vi "Get Context.vi"(8 "error in":errorcluster) -> (0 "error out":errorcluster, 3 "context":refnum<class "zmq_context.lvclass">)   [LabVIEW 2019, in "RemoteControl.ZMQ.lvlib" / "ZMQ.ContextManager.lvlib"]
uses:
  ZMQ.ContextManager.lvlib
  <vilib>/addons/zeromq/zmq_context.lvclass
  Typedefs/Action--enum.ctl
  private/Context Owner.vi
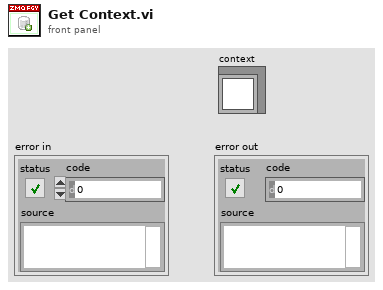
[diagram p1: front panel]
types:
  T1 = typedef "RemoteControl.ZMQ.lvlib/ZMQ.ContextManager.lvlib/Action--enum.ctl" = enum16{"Get Context", "Release Context", "Socket Opened", "Socket Closed", "Force Cleanup", "Set Context", "Retire If Idle"}
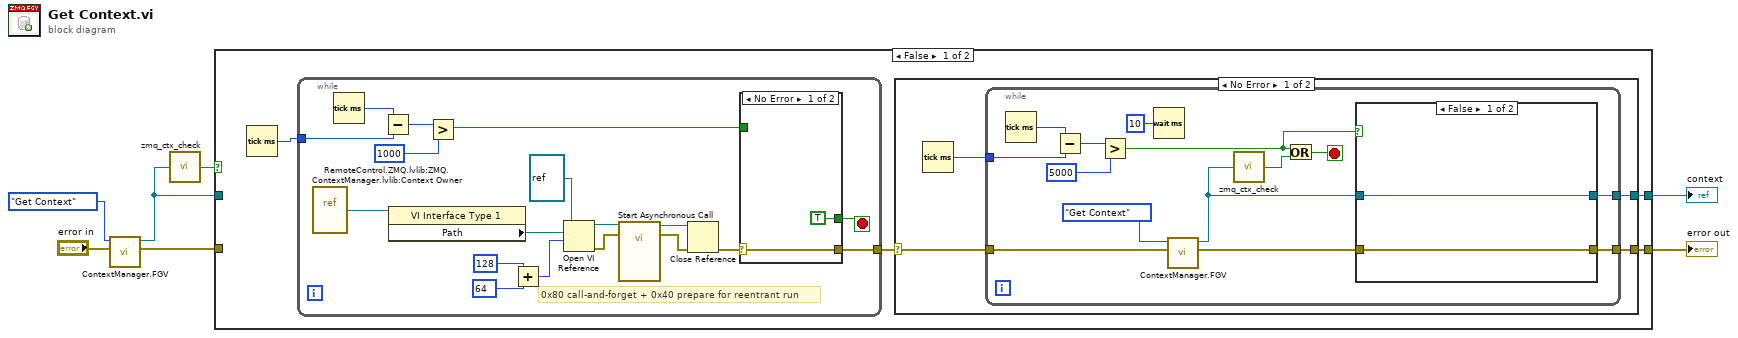
[diagram p0: block diagram]
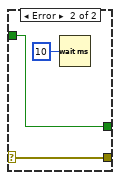
[diagram p2: hidden frame]
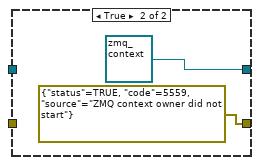
[diagram p3: hidden frame]
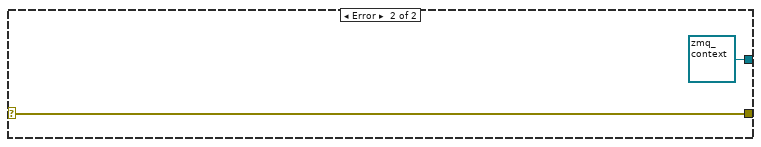
[diagram p4: hidden frame]
diagram:
  n1 = call "ContextManager.FGV.vi"("error in"="error in", "action"=Action--enum."Get Context") -> ("error out"=w1:errorcluster, "context out"=w2:refnum<class "zmq_context.lvclass">)  [unwired: 7 in, 1 out]
  n2 = call <vilib>:"zmq_ctx_check.vi"("context in"=w2) -> ("valid?"=w3:bool)
  n3 = case shown="False" w3 {
    tunnel: w2 -> [_ w60]
    tunnel: [w11 w60] -> w5
    tunnel: [w10 w59] -> w4
    tunnel: w1 -> [_ w59]
    frame False {
      n4 = Tick Count (ms)() -> (millisecond timer value=w9:u32)
      n5 = while {
        tunnel: w9 -> [w19]
        tunnel: [w15] -> w8
        stop <- w16 stop-if-true
        # "0x80 call-and-forget + 0x40 prepare for reentrant run"
        n6 = vi-ref "RemoteControl.ZMQ.lvlib:ZMQ.ContextManager.lvlib:Context Owner.vi"() -> (w24:refnum<vi>)
        n7 = Tick Count (ms)() -> (millisecond timer value=w20:u32)
        n8 = Subtract(x=w20, y=w19) -> (x-y=w21:u32)
        n9 = property class="VI Interface Type 1"(reference=w24) -> ("Path"=w25:path)  [unwired: 1 in, 2 out]
        n10 = Greater?(x=w21, y=u32 1000) -> (0:w17:bool)
        n11 = Add(x=128 ("options"), y=64 ("options")) -> (x+y=w12:i32)
        n12 = Open VI Reference(type specifier VI Refnum (for type only)=refnum<vi> refnum, vi path=w25, options=w12) -> (vi reference=w23:refnum<vi>, error out=w29:errorcluster)  [unwired: 3 in]
        n13 = call-by-ref "Start Asynchronous Call"(reference=w23, error in=w29) -> (reference out=w28:refnum<vi>, error out=w27:errorcluster)  [unwired: 1 in]
        n14 = Close Reference(reference=w28, error in (no error)=w27) -> (error out=w18:errorcluster)
        n15 = case shown="No Error" w18 {
          selector: w18 -> [w30 w32]
          tunnel: w17 -> [_ w33]
          tunnel: [TRUE w33] -> w16
          tunnel: [w30 w32] -> w15
          frame No Error {
          }
          frame Error {
            n16 = Wait (ms)(milliseconds to wait=u32 10) -> ()  [unwired: 1 out]
          }
        }
      }
      n17 = case shown="No Error" w8 {
        selector: w8 -> [w35 w57]
        tunnel: [w37 refnum<class "zmq_context.lvclass"> refnum ("context")] -> w11
        tunnel: [w36 w57] -> w10
        frame No Error {
          n18 = Tick Count (ms)() -> (millisecond timer value=w38:u32)
          n19 = while {
            tunnel: w35 -> [w49]
            tunnel: w38 -> [w51]
            tunnel: [w44] -> w37
            tunnel: [w43] -> w36
            stop <- w48 stop-if-true
            n20 = Tick Count (ms)() -> (millisecond timer value=w52:u32)
            n21 = Subtract(x=w52, y=w51) -> (x-y=w47:u32)
            n22 = Greater?(x=w47, y=u32 5000) -> (0:w45:bool)
            n23 = Wait (ms)(milliseconds to wait=u32 10) -> ()  [unwired: 1 out]
            n24 = call "ContextManager.FGV.vi"("error in"=w49, "action"=Action--enum."Get Context") -> ("error out"=w42:errorcluster, "context out"=w41:refnum<class "zmq_context.lvclass">)  [unwired: 7 in, 1 out]
            n25 = call <vilib>:"zmq_ctx_check.vi"("context in"=w41) -> ("valid?"=w40:bool)
            n26 = Or(x=w45, y=w40) -> (x .or. y?=w48:bool)
            n27 = case shown="False" w45 {
              tunnel: [w53 refnum<class "zmq_context.lvclass"> refnum ("context")] -> w44
              tunnel: [w54 errorcluster {"status"=TRUE, "code"=5559, "source"="ZMQ context owner did not start"} ("error out")] -> w43
              tunnel: w42 -> [w54 _]
              tunnel: w41 -> [w53 _]
              frame False {
              }
              frame True {
              }
            }
          }
        }
        frame Error {
        }
      }
    }
    frame True {
    }
  }
  "error out" <- w4
  "context" <- w5
